vi "shm info init.vi"(8 "error in (no error)":errorcluster, 10 "shared memory configuration in":refnum<class "Shared Memory configuration.lvclass">, 11 "shared memory runtime in":refnum<class "Shared Memory runtime.lvclass">) -> (0 "error out":errorcluster, 2 "shared memory configuration out":refnum<class "Shared Memory configuration.lvclass">, 3 "shared memory runtime out":refnum<class "Shared Memory runtime.lvclass">)   [LabVIEW 2014, in "Shared Memory runtime.lvclass"]
uses:
  Shared Memory runtime.lvclass
  configuration/Shared Memory configuration.lvclass
  controls/shm info.ctl
  <vilib>/NI/NI Linux RT IPC/Shared Memory/Controls/reference.ctl
  <vilib>/NI/NI Linux RT IPC/Shared Memory/Classes/Shared Memory/Shared Memory.lvclass
  controls/shm info ptrs.ctl
  configuration/Shared Memory configuration.lvclass/Shared Memory configuration.ctl
  Shared Memory runtime.lvclass/Shared Memory runtime.ctl
  <vilib>/NI/NI Linux RT IPC/Shared Memory/Pointer Operations/Write Scalar U16.vi
  configuration/Read engine info shm name.vi
  configuration/Read revision major.vi
  configuration/Read header minor.vi
  configuration/Read revision fix.vi
  configuration/Read revision build.vi
  Write shm info.vi
  <vilib>/NI/NI Linux RT IPC/Shared Memory/Linux RT IPC.Shared Memory.lvlib
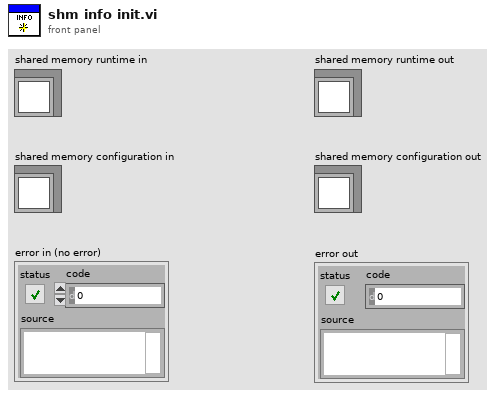
[diagram p1: front panel]
types:
  T1 = typedef "Shared Memory runtime.lvclass/shm info.ctl" = cluster{"shared memory":T2, "shm info ptrs":T3, "created?":bool}
  T2 = typedef "Linux RT IPC.Shared Memory.lvlib/reference.ctl" = refnum<data-value>
  T3 = typedef "Shared Memory runtime.lvclass/shm info ptrs.ctl" = cluster{"rev_major_ptr":u64, "rev_minor_ptr":u64, "rev_fix_ptr":u64, "rev_build_ptr":u64}
  T4 = cluster{"owner":cluster{"read":bool, "write":bool, "execute":bool}, "group":cluster{"read":bool, "write":bool, "execute":bool}, "everyone":cluster{"read":bool, "write":bool, "execute":bool}}
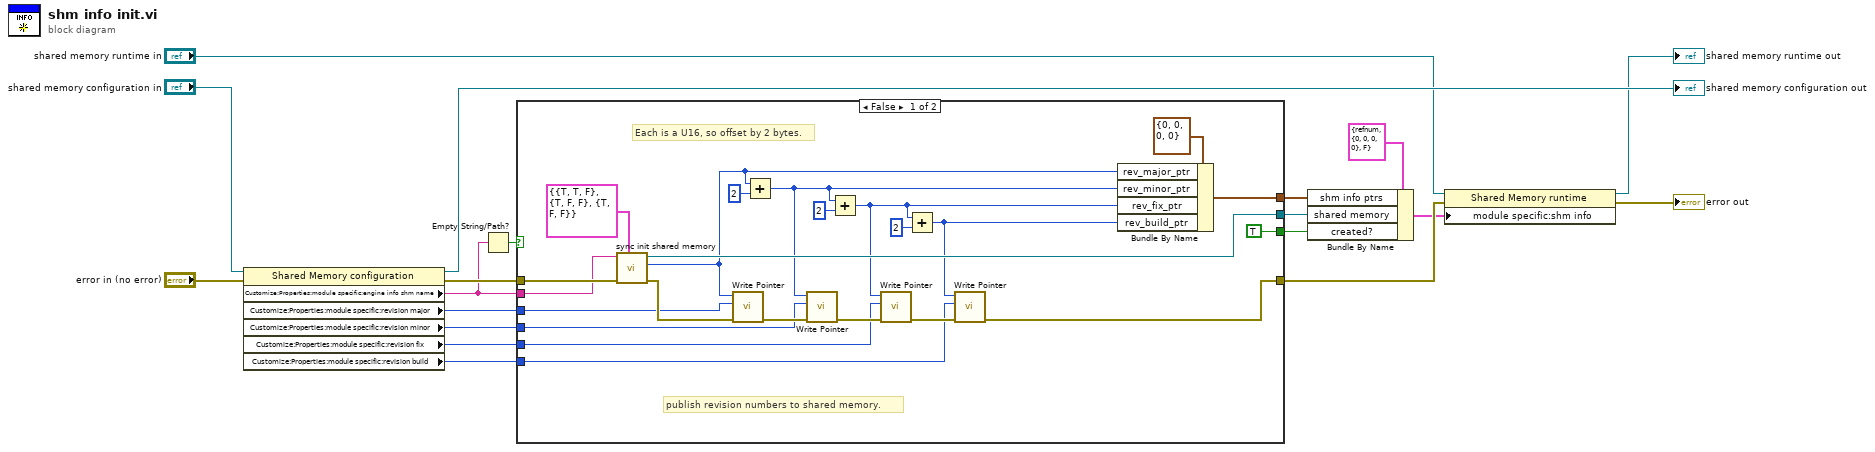
[diagram p0: block diagram]
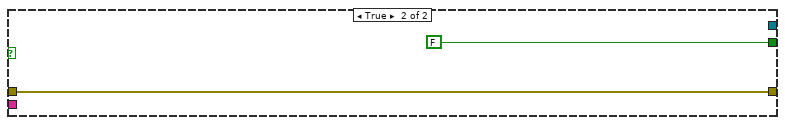
[diagram p2: hidden frame]
diagram:
  n1 = property class="Shared Memory configuration"(reference="shared memory configuration in", error in="error in (no error)") -> (reference out=→"shared memory configuration out":refnum<class "Shared Memory configuration.lvclass">, error out=w13:errorcluster, "Customize:Properties:module specific:engine info shm name"=w5:string, "Customize:Properties:module specific:revision major"=w9:u16, "Customize:Properties:module specific:revision minor"=w6:u16, "Customize:Properties:module specific:revision fix"=w2:u16, "Customize:Properties:module specific:revision build"=w1:u16)
  n2 = Empty String/Path?(string/path=w5) -> (empty?=w4:bool)
  n3 = case shown="False" w4 {
    tunnel: w13 -> [w42 w44]
    tunnel: w5 -> [w41 _]
    tunnel: [w38 _] -> w11
    tunnel: [w37 _] -> w10
    tunnel: w9 -> [w35 _]
    tunnel: [w25 w44] -> w8
    tunnel: w6 -> [w33 _]
    tunnel: [TRUE FALSE] -> w3
    tunnel: w2 -> [w21 _]
    tunnel: w1 -> [w20 _]
    frame False {
      # "publish revision numbers to shared memory."
      # "Each is a U16, so offset by 2 bytes."
      n4 = call "sync init shared memory.vi"("permissions (0664)"=T4 {"owner"={"read"=TRUE, "write"=TRUE, "execute"=FALSE}, "group"={"read"=TRUE, "write"=FALSE, "execute"=FALSE}, "everyone"={"read"=TRUE, "write"=FALSE, "execute"=FALSE}}, "error in (no error)"=w42, "sync shm name"=w41) -> ("error out"=w36:errorcluster, "pointer to shared memory"=w22:u64, "shared memory out"=w38:T2)  [unwired: 6 in]
      n5 = call-poly <vilib>:"Write Pointer.vi"("error in (no error)"=w36, "value"=w35, "pointer in"=w22) -> ("error out"=w34:errorcluster)  [unwired: 7 in, 1 out]
      n6 = Add(x=w22, y=u64 2) -> (x+y=w28:u64)
      n7 = call-poly <vilib>:"Write Pointer.vi"("error in (no error)"=w34, "value"=w33, "pointer in"=w28) -> ("error out"=w27:errorcluster)  [unwired: 7 in, 1 out]
      n8 = Add(x=w28, y=u64 2) -> (x+y=w24:u64)
      n9 = call-poly <vilib>:"Write Pointer.vi"("error in (no error)"=w27, "value"=w21, "pointer in"=w24) -> ("error out"=w26:errorcluster)  [unwired: 7 in, 1 out]
      n10 = Add(x=w24, y=u64 2) -> (x+y=w23:u64)
      n11 = call-poly <vilib>:"Write Pointer.vi"("error in (no error)"=w26, "value"=w20, "pointer in"=w23) -> ("error out"=w25:errorcluster)  [unwired: 7 in, 1 out]
      n12 = Bundle By Name(cluster=T3 {"rev_major_ptr"=0, "rev_minor_ptr"=0, "rev_fix_ptr"=0, "rev_build_ptr"=0} ("shm info ptrs"), "rev_major_ptr"=w22, "rev_minor_ptr"=w28, "rev_fix_ptr"=w24, "rev_build_ptr"=w23) -> (w37:T3)
    }
    frame True {
    }
  }
  n13 = Bundle By Name(cluster=T1 {"shared memory"=refnum, "shm info ptrs"={"rev_major_ptr"=0, "rev_minor_ptr"=0, "rev_fix_ptr"=0, "rev_build_ptr"=0}, "created?"=FALSE} ("shm info"), "shm info ptrs"=w10, "shared memory"=w11, "created?"=w3) -> (w7:T1)
  n14 = property class="Shared Memory runtime"(reference="shared memory runtime in", error in=w8, "module specific:shm info"=w7) -> (reference out=→"shared memory runtime out":refnum<class "Shared Memory runtime.lvclass">, error out=→"error out":errorcluster)
